vi "Check Action.vi"(6 "HRS Time":dbl, 7 "Values In":dbl[](array[numeric]), 8 "error in (no error)":errorcluster, 11 "SequencedValves in":refnum<class "SeqDelayControl.lvclass">) -> (0 "error out":errorcluster, 2 "Actions":T1[](array[typedef]), 3 "SequencedValves out":refnum<class "SeqDelayControl.lvclass">, 5 "Values":dbl[](array[numeric]))   [LabVIEW 2020, in "VolatusControl.lvlib" / "SeqDelayControl.lvclass"]
uses:
  SeqDelayControl.lvclass
  Control Action.ctl
  SeqDelayControl.lvclass/SeqDelayControl.ctl
  State.ctl
  Volatus/MessageQ/MessageQ.lvclass
  VolatusControl.lvlib
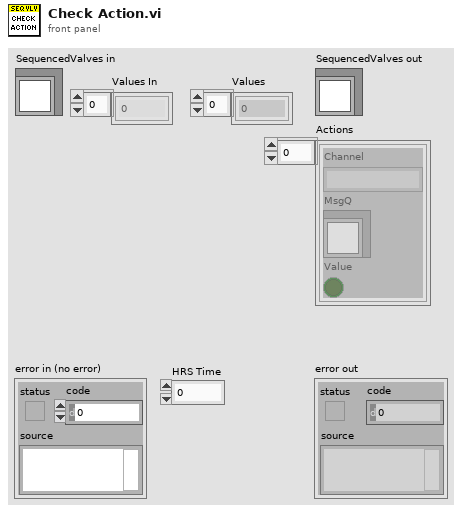
[diagram p1: front panel]
types:
  T1 = typedef "VolatusControl.lvlib/Control Action.ctl" = cluster{"Channel":string, "MsgQ":refnum<class "MessageQ.lvclass">, "Value":bool}
  T2 = typedef "VolatusControl.lvlib/SeqDelayControl.lvclass/State.ctl" = enum16{"Idle", "Start", "Delay"}
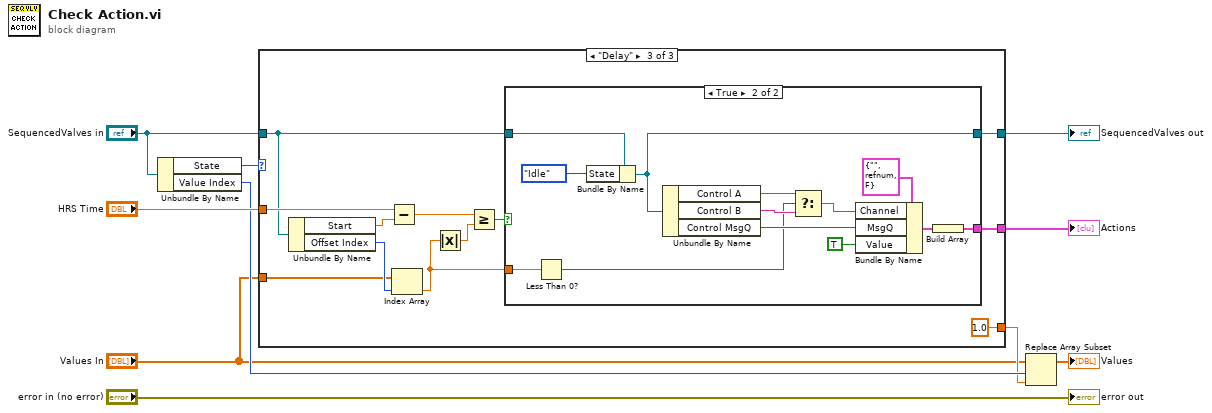
[diagram p0: block diagram]
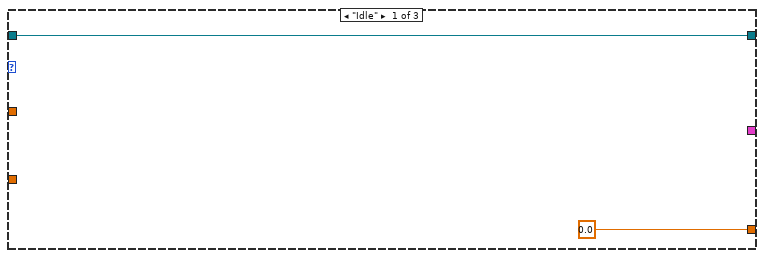
[diagram p2: hidden frame]
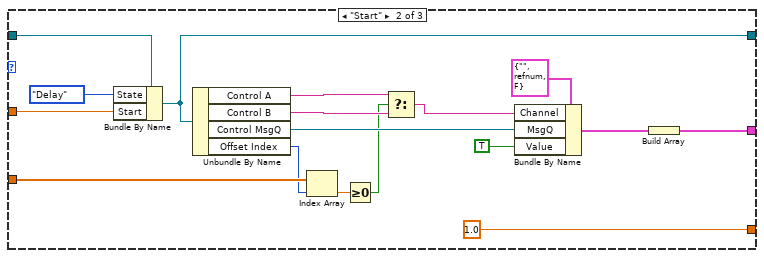
[diagram p3: hidden frame]
diagram:
  n1 = Unbundle By Name("SequencedValves in") -> ("State"=w9:T2, "Value Index"=w3:i32)
  n2 = case shown="\"Delay\"" w9 {
    tunnel: "SequencedValves in" -> [w12 w26 w37]
    tunnel: "HRS Time" -> [_ w24 w41]
    tunnel: [w12 w23 w36] -> w6
    tunnel: [_ w13 w35] -> w5
    tunnel: [0.0 1.0 1.0] -> w2
    tunnel: "Values In" -> [_ w20 w33]
    frame "Idle" {
    }
    frame "Start" {
      n3 = Bundle By Name(cluster=w26, "State"=State."Delay", "Start"=w24) -> (w23:refnum<class "SeqDelayControl.lvclass">)
      n4 = Unbundle By Name(w23) -> ("Control A"=w16:string, "Control B"=w17:string, "Control MsgQ"=w22:refnum<class "MessageQ.lvclass">, "Offset Index"=w19:i32)
      n5 = Index Array(array=w20, index=w19) -> (element=w18:dbl)
      n6 = Greater Or Equal To 0?(x=w18) -> (x >= 0?=w15:bool)
      n7 = Select(t=w16, s=w15, f=w17) -> (s? t:f=w14:string)
      n8 = Bundle By Name(cluster=T1 {"Channel"="", "MsgQ"=refnum, "Value"=FALSE} ("Action"), "Channel"=w14, "MsgQ"=w22, "Value"=TRUE) -> (w28:T1)
      n9 = Build Array(w28) -> (w13:T1[])
    }
    frame "Delay" {
      n10 = Unbundle By Name(w37) -> ("Start"=w40:dbl, "Offset Index"=w34:i32)
      n11 = Subtract(x=w41, y=w40) -> (x-y=w39:dbl)
      n12 = Index Array(array=w33, index=w34) -> (element=w30:dbl)
      n13 = Absolute Value(x=w30) -> (abs(x)=w31:dbl)
      n14 = Greater Or Equal?(x=w39, y=w31) -> (x >= y?=w38:bool)
      n15 = case shown="True" w38 {
        tunnel: w37 -> [w42 w51]
        tunnel: [w42 w50] -> w36
        tunnel: [_ w43] -> w35
        tunnel: w30 -> [_ w46]
        frame False {
        }
        frame True {
          n16 = Less Than 0?(x=w46) -> (x < 0?=w45:bool)
          n17 = Bundle By Name(cluster=w51, "State"=State."Idle") -> (w50:refnum<class "SeqDelayControl.lvclass">)
          n18 = Unbundle By Name(w50) -> ("Control A"=w48:string, "Control B"=w47:string, "Control MsgQ"=w53:refnum<class "MessageQ.lvclass">)
          n19 = Select(t=w48, s=w45, f=w47) -> (s? t:f=w44:string)
          n20 = Bundle By Name(cluster=T1 {"Channel"="", "MsgQ"=refnum, "Value"=FALSE} ("Action"), "Channel"=w44, "MsgQ"=w53, "Value"=TRUE) -> (w52:T1)
          n21 = Build Array(w52) -> (w43:T1[])
        }
      }
    }
  }
  "SequencedValves out" <- w6
  "Actions" <- w5
  n22 = Replace Array Subset(array="Values In", new element=w2, index=w3) -> (→"Values":dbl[])
  "error out" <- "error in (no error)"
